vi "Lookup Object Hierarchy.vi"(8 "error in (no error)":errorcluster, 10 "LabVIEW Object":refnum<class>) -> (0 "error out":errorcluster, 1 "Library Versions":T1(array[cluster]), 2 "Private Data Clusters":variant[](array[variant]), 3 "Class Names":string[](array[string]))   [LabVIEW 2017, in "Composition.lvlib"]
doc: "Returns the private data clusters and version numbers for all classes in the object hierarchy in ascending order (most specific children first).\n\n<B>Note</B> This operation is very slow, which is why this VI holds a lookup table in memory to improve performance considerably."
uses:
  Composition.lvlib
  <vilib>/Utility/EditLVLibs/Edit LVLibs.lvlib
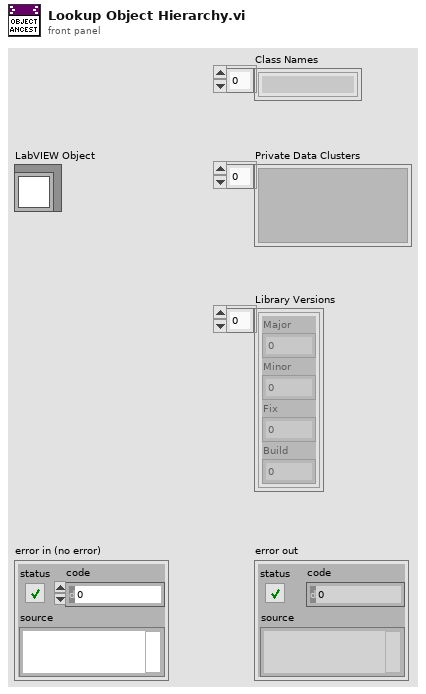
[diagram p1: front panel]
types:
  T1 = cluster{"Major":u16, "Minor":u16, "Fix":u16, "Build":u16}[]
  T2 = cluster{cluster{"Major":u16, "Minor":u16, "Fix":u16, "Build":u16}[]}[]
  T3 = typedef "Edit LVLibs.lvlib/LibVersion.ctl" = cluster{"Major":u16, "Minor":u16, "Fix":u16, "Build":u16}
  T4 = typedef "Edit LVLibs.lvlib/Mutation History.ctl" = T5[]
  T5 = typedef "Edit LVLibs.lvlib/Mutation Record.ctl" = cluster{"Library Version":T3, "Old Name Index":u8, "Class Default Data":variant, "Cluster Order Map":u32[], "Parent Name":string, "Parent Path":path, "LabVIEW Version":u32, "User Comments":string, "Mutation Flags":u8, "Parent Old Name Index":u8, "Parent Levels Added":u16, "Parent Levels Removed":u16}
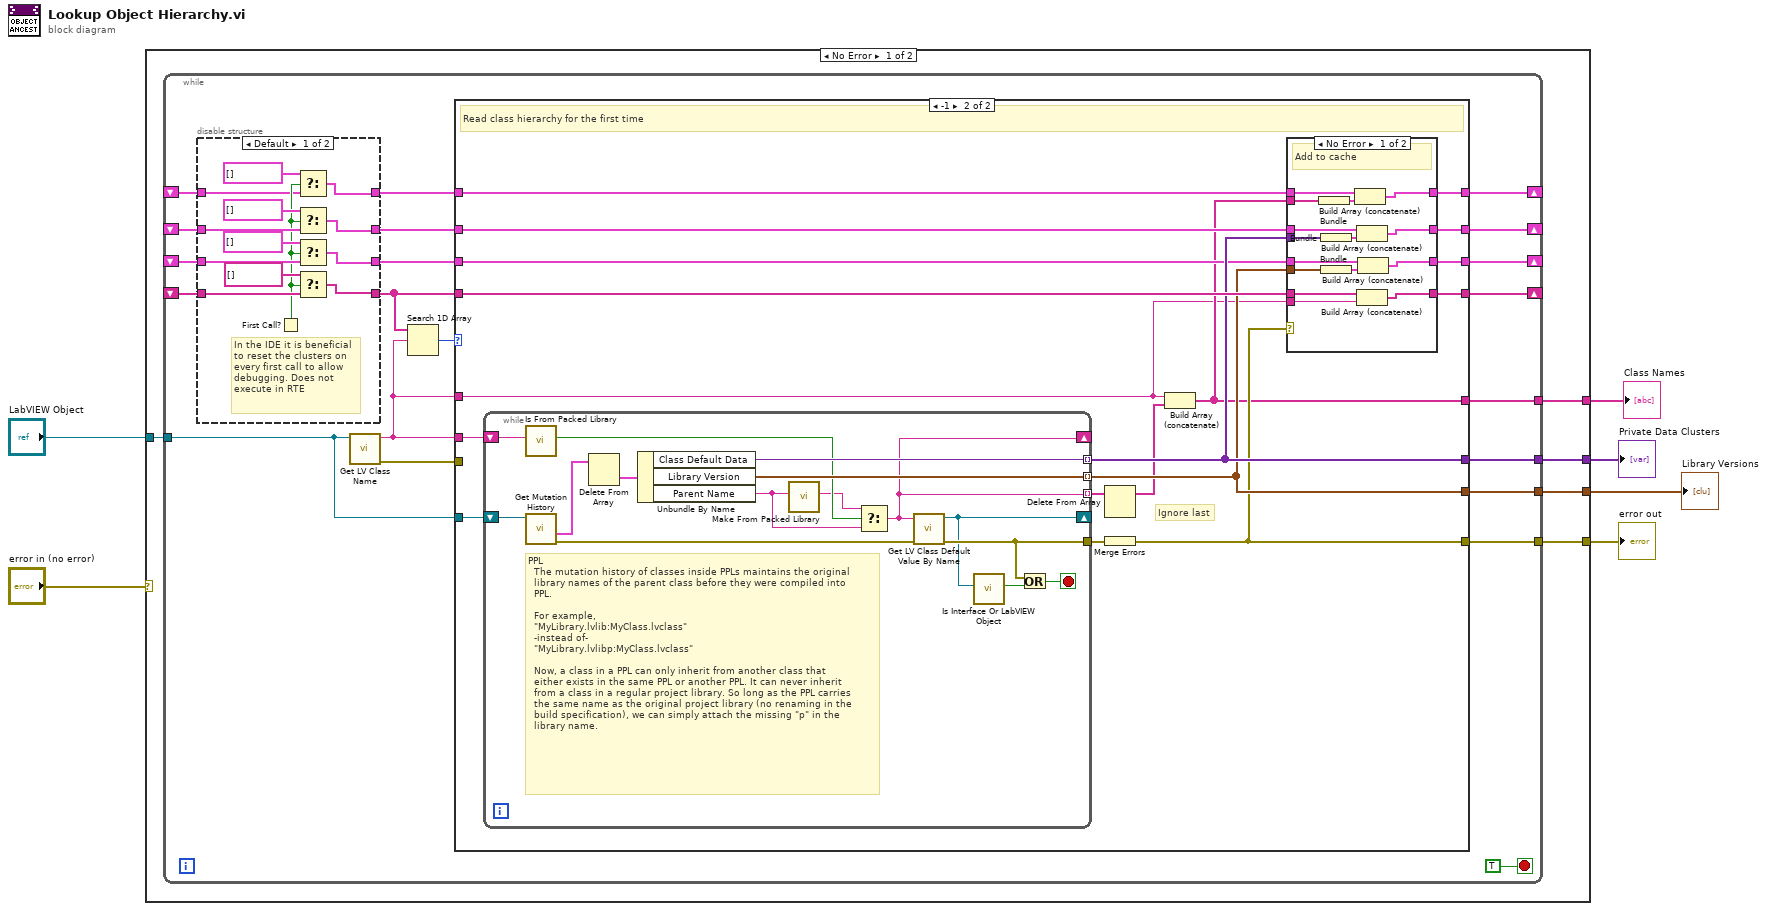
[diagram p0: block diagram]
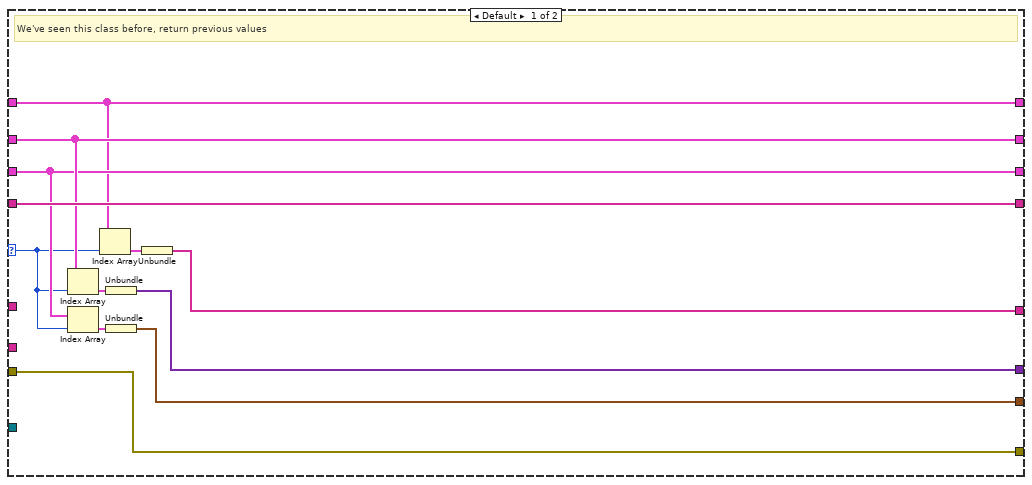
[diagram p2: hidden frame]
diagram:
  n1 = case shown="No Error" "error in (no error)" {
    selector: "error in (no error)" -> [_ w114]
    tunnel: "LabVIEW Object" -> [w11 _]
    tunnel: [w10 _] -> w5
    tunnel: [w9 w114] -> w3
    tunnel: [w8 _] -> w2
    tunnel: [w7 _] -> w1
    frame No Error {
      n2 = while {
        tunnel: w11 -> [w13]
        tunnel: [w32] -> w10
        tunnel: [w31] -> w9
        shift-right: [w29] -> _
        shift-left: _ -> [w23]
        shift-right: [w27] -> _
        shift-left: _ -> [w19]
        shift-right: [w26] -> _
        shift-left: _ -> [w21]
        tunnel: [w25] -> w8
        tunnel: [w17] -> w7
        shift-right: [w15] -> _
        shift-left: _ -> [w16]
        stop <- TRUE stop-if-true
        n3 = disable-structure shown="Default" {
          disable-tunnel: [w108 w113] -> w24
          disable-tunnel: w23 -> [w109 w113]
          disable-tunnel: [w104 w112] -> w22
          disable-tunnel: w21 -> [w107 w112]
          disable-tunnel: [w105 w111] -> w20
          disable-tunnel: w19 -> [w106 w111]
          disable-tunnel: w16 -> [w99 w110]
          disable-tunnel: [w98 w110] -> w14
          frame condition #0 (active) {
            # "In the IDE it is beneficial\nto reset the clusters on\nevery first call to allow\ndebugging. Does not\nexecute in RTE"
            n4 = First Call?() -> (First Call?: T/F=w100:bool)
            n5 = Select(t=cluster{string[]}[] [], s=w100, f=w99) -> (s? t:f=w98:cluster{string[]}[])
            n6 = Select(t=cluster{variant[]}[] [], s=w100, f=w109) -> (s? t:f=w108:cluster{variant[]}[])
            n7 = Select(t=T2 [], s=w100, f=w107) -> (s? t:f=w104:cluster{T3[]}[])
            n8 = Select(t=string[] [], s=w100, f=w106) -> (s? t:f=w105:string[])
          }
          frame condition #1 {
          }
        }
        n9 = call <vilib>:"Get LV Class Name.vi"("object"=w13) -> ("error out"=w18:errorcluster, "class name"=w12:string)  [unwired: 9 in]
        n10 = Search 1D Array(1D array=w20, element=w12) -> (index of element=w28:i32)  [unwired: 1 in]
        n11 = case shown="-1" w28 {
          selector: w28 -> [w35 _]
          tunnel: w12 -> [_ w48]
          tunnel: [w40 w58] -> w32
          tunnel: [w43 w52] -> w31
          tunnel: w24 -> [w42 w61]
          tunnel: w18 -> [w43 _]
          tunnel: [w42 w62] -> w29
          tunnel: w20 -> [w44 w60]
          tunnel: [w44 w59] -> w27
          tunnel: [w37 w55] -> w25
          tunnel: w22 -> [w38 w57]
          tunnel: [w38 w56] -> w26
          tunnel: [w33 w50] -> w17
          tunnel: [w34 w54] -> w15
          tunnel: w14 -> [w34 w53]
          tunnel: w13 -> [_ w49]
          tunnel: w12 -> [_ w45]
          frame Default {
            # "We've seen this class before, return previous values"
            n12 = Index Array(array=w42, index=w35) -> (element=w41:cluster{variant[]})
            n13 = Index Array(array=w38, index=w35) -> (element=w39:cluster{T3[]})
            n14 = Index Array(array=w34, index=w35) -> (element=w36:cluster{string[]})
            n15 = Unbundle(w41) -> (w40:variant[])
            n16 = Unbundle(w39) -> (w37:T3[])
            n17 = Unbundle(w36) -> (w33:string[])
          }
          frame -1 {
            # "Ignore last"
            # "Read class hierarchy for the first time"
            n18 = while {
              tunnel: [w71] -> w58 mode=indexing
              tunnel: [w72] -> w55 mode=indexing
              tunnel: [w73] -> w51
              shift-right: [w69] -> _
              shift-left: w49 -> [w75]
              tunnel: [w63] -> w47 mode=indexing
              shift-right: [w63] -> _
              shift-left: w45 -> [w67]
              stop <- w70 stop-if-true
              # "PPL\n  The mutation history of classes inside PPLs maintains the original\n  library names of the parent class before they were compiled into\n  PPL.\n\n  For example,\n  \"MyLibrary.lvlib:MyClass.lvclass\"\n  -instead of-\n  \"MyLibrary.lvlibp:MyClass.lvclass\"\n  \n  Now, a class in a PPL can only inherit from another class that\n  either exists in the same PPL or another PPL. It can never inherit\n  from a class in a regular project library. So long as the PPL carries\n  the same name as the original project library (no renaming in the\n  build specification), we can simply attach the missing \"p\" in the\n  library name."
              n19 = call "Is From Packed Library.vi"("Qualified Name"=w67) -> ("Is From Packed Library"=w66:bool)  [unwired: 10 in]
              n20 = call <vilib>:"Get Mutation History.vi"("Input object"=w75) -> ("error out"=w74:errorcluster, "Mutation History"=w76:T4)  [unwired: 7 in]
              n21 = Delete From Array(array=w76) -> (deleted portion=w77:T5)  [unwired: 2 in, 1 out]
              n22 = Unbundle By Name(w77) -> ("Class Default Data"=w71:variant, "Library Version"=w72:T3, "Parent Name"=w64:string)
              n23 = call "Make From Packed Library.vi"("Fully Qualified String"=w64) -> ("Fully Qualified String out"=w65:string)  [unwired: 10 in]
              n24 = Select(t=w65, s=w66, f=w64) -> (s? t:f=w63:string)
              n25 = call <vilib>:"Get LV Class Default Value By Name.vi"("error in (no error)"=w74, "class name"=w63) -> ("error out"=w73:errorcluster, "object"=w69:refnum<class>)  [unwired: 8 in]
              n26 = call "Is Interface Or LabVIEW Object.vi"("LabVIEW Object"=w69) -> ("Is Interface Or LabVIEW Object"=w68:bool)  [unwired: 10 in]
              n27 = Or(x=w73, y=w68) -> (x .or. y?=w70:bool)
            }
            n28 = Delete From Array(array=w47) -> (array with subset deleted=w46:string[])  [unwired: 2 in, 1 out]
            n29 = Merge Errors(w51) -> (w52:errorcluster)
            n30 = Build Array (concatenate)(w48, w46) -> (w50:string[])
            n31 = case shown="No Error" w52 {
              tunnel: [w92 w95] -> w62
              tunnel: w61 -> [w91 w95]
              tunnel: w60 -> [w90 w93]
              tunnel: w48 -> [w89 _]
              tunnel: [w88 w93] -> w59
              tunnel: w58 -> [w87 _]
              tunnel: w57 -> [w85 w94]
              tunnel: [w84 w94] -> w56
              tunnel: w55 -> [w83 _]
              tunnel: [w80 w96] -> w54
              tunnel: w50 -> [w79 _]
              tunnel: w53 -> [w78 w96]
              frame No Error {
                # "Add to cache"
                n32 = Bundle(w79) -> (w81:cluster{string[]})  [unwired: 1 in]
                n33 = Bundle(w87) -> (w86:cluster{variant[]})  [unwired: 1 in]
                n34 = Bundle(w83) -> (w82:cluster{T3[]})  [unwired: 1 in]
                n35 = Build Array (concatenate)(w78, w81) -> (w80:cluster{string[]}[])
                n36 = Build Array (concatenate)(w91, w86) -> (w92:cluster{variant[]}[])
                n37 = Build Array (concatenate)(w90, w89) -> (w88:string[])
                n38 = Build Array (concatenate)(w85, w82) -> (w84:cluster{T3[]}[])
              }
              frame Error {
                # "Don't cache"
              }
            }
          }
        }
      }
    }
    frame Error {
    }
  }
  "Private Data Clusters" <- w5
  "error out" <- w3
  "Library Versions" <- w2
  "Class Names" <- w1
